vi "Power On Dut.vi"(7 "measure call context in":refnum<class "Measure Call Context.lvclass">, 8 "error in":errorcluster, 11 "Power sequencing file path":path) -> (0 "error out":errorcluster, 5 "measure call context out":refnum<class "Measure Call Context.lvclass">)   [LabVIEW 2023]
uses:
  <vilib>/Plug-In SDKs/Measurements/Measure Call Context/Measure Call Context.lvclass
  NI gRPC Device Server - Action.ctl
  <instrlib>/niDCPower/nidcpower.llb/niDCPower gRPC Device Server.ctl
  <instrlib>/niDCPower/nidcpower.llb/niDCPower Source Mode.ctl
  <instrlib>/niDCPower/nidcpower.llb/niDCPower Output Function.ctl
  <instrlib>/niDigital/niDigital.llb/niDigital gRPC Device Server.ctl
  <instrlib>/niDigital/niDigital.llb/niDigital Output Function.ctl
  <instrlib>/niDigital/niDigital.llb/niDigital PMU Aperture Time Units.ctl
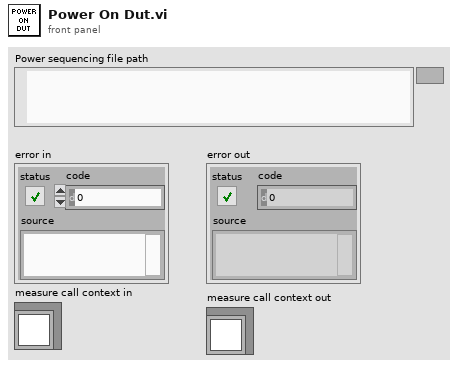
[diagram p1: front panel]
types:
  T1 = typedef "NI gRPC Device Server - Action.ctl" = enum16{"Start Server", "End Server"}
  T2 = typedef "DC Ins Initialize.ctl" = cluster{"Pin Name":string, "Resource Name":refnum<k15>, "Channel":string, "Voltage Range (V)":dbl, "Current Range (A)":dbl, "Instrument Type":T3}
  T3 = typedef "DC Ins Type.ctl" = enum16{"niDigital", "niDCPower", "undefined"}
  T4 = typedef "DC Settings.ctl" = cluster{"Pin Name":string, "Resource Name":refnum<k15>, "Channel":string, "Power-up Seq":u32, "Power-up Voltage (V)":dbl, "Power-down Seq":u32, "Power-down Voltage (V)":dbl, "Current Limit (A)":dbl, "Wait Before Next (ms)":u32, "Instrument Type":T3}
  T5 = typedef "niDCPower gRPC Device Server.ctl" = cluster{"session name":string, "address (localhost)":string, "port (31763)":u32}
  T6 = typedef "niDigital gRPC Device Server.ctl" = cluster{"session name":string, "address (localhost)":string, "port (31763)":u32}
  T7 = typedef "niDCPower Output Function.ctl" = i32
  T8 = typedef "niDCPower Source Mode.ctl" = i32
  T9 = typedef "niDigital PMU Aperture Time Units.ctl" = i32
  T10 = typedef "niDigital Output Function.ctl" = i32
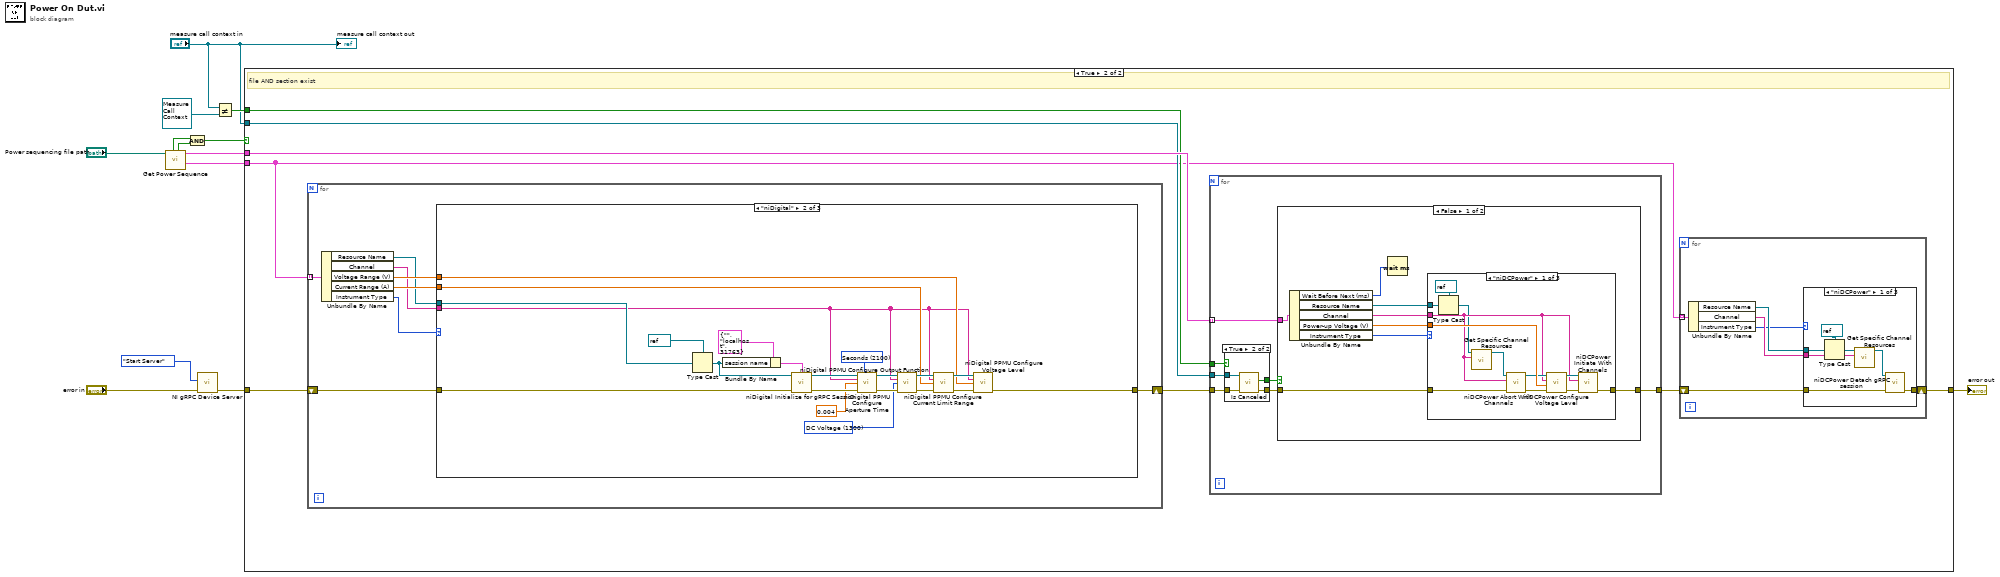
[diagram p0: block diagram]
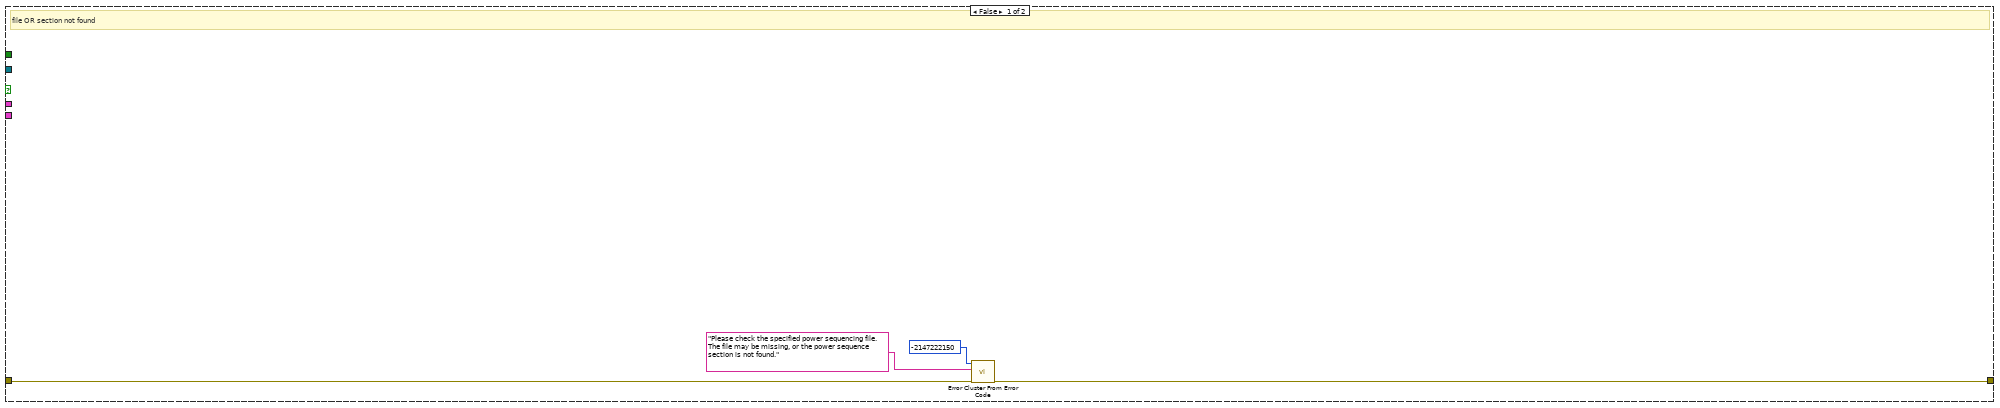
[diagram p2: hidden frame]
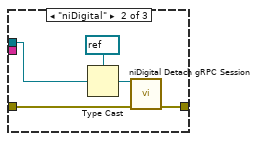
[diagram p3: hidden frame]
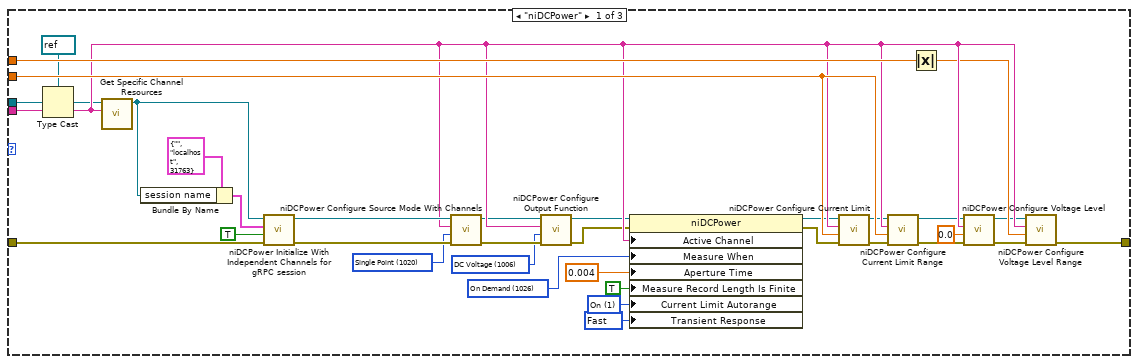
[diagram p5: hidden frame]
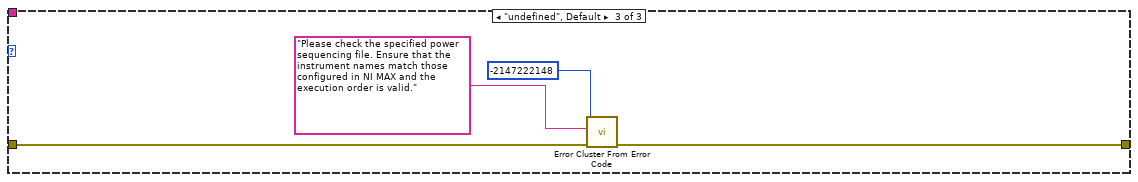
[diagram p6: hidden frame]
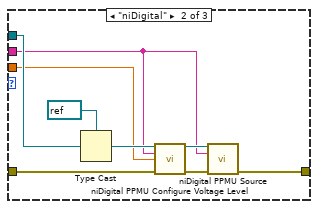
[diagram p8: hidden frame]
diagram:
  n1 = call "Get Power Sequence.vi"("File Path"="Power sequencing file path") -> ("SMUs to Initialize (not in order)"=w12:T2[], "Power up Seq"=w11:T4[], "File Exists?"=w7:bool, "Section Exists?"=w6:bool)  [unwired: 6 in, 1 out]
  n2 = And(x=w6, y=w7) -> (x .and. y?=w8:bool)
  n3 = call "NI gRPC Device Server.vi"("error in"="error in", "Action"=NI_gRPC_Device_Server_-_Action."Start Server") -> ("error out"=w5:errorcluster)  [unwired: 9 in]
  n4 = Not Equal?(x="measure call context in", y=refnum<class "Measure Call Context.lvclass"> refnum ("measure call context in")) -> (x != y?=w4:bool)
  n5 = case shown="True" w8 {
    tunnel: w12 -> [_ w18]
    tunnel: w11 -> [_ w25]
    tunnel: [w17 w21] -> w10
    tunnel: w5 -> [w16 w23]
    tunnel: "measure call context in" -> [_ w20]
    tunnel: w4 -> [_ w19]
    frame False {
      # "file OR section not found"
      n6 = call <vilib>:"Error Cluster From Error Code.vi"("error in (no error)"=w16, "error message (\"\")"="Please check the specified power sequencing file. The file may be missing, or the power sequence section is not found.", "error code (0)"=-2147222150) -> ("error out"=w17:errorcluster)  [unwired: 6 in]
    }
    frame True {
      # "file AND section exist"
      n7 = for {
        tunnel: w18 -> [w51] mode=indexing
        shift-right: [w47] -> w24
        shift-left: w23 -> [w52]
        n8 = Unbundle By Name(w51) -> ("Resource Name"=w46:refnum<k15>, "Channel"=w48:string, "Voltage Range (V)"=w50:dbl, "Current Range (A)"=w49:dbl, "Instrument Type"=w45:T3)
        n9 = case shown="\"niDigital\"" w45 {
          tunnel: w46 -> [w87 w91 _]
          tunnel: w52 -> [w86 w108 w112]
          tunnel: w50 -> [w85 w90 _]
          tunnel: w49 -> [w84 w89 _]
          tunnel: w48 -> [w76 w88 _]
          tunnel: [w83 w107 w111] -> w47
          frame "niDCPower" {
            w53 = 1039 items=["Slow"=1041, "Normal"=1038, "Fast"=1039, "Custom"=1042] ("Source:Transient Response")
            w54 = 1 items=["Off", "On"] ("Measurement:Autorange")
            w69 = 1026 items=["Automatically after Source Complete"=1025, "On Demand"=1026, "On Measure Trigger"=1027] ("Measurement:Advanced:Measure When")
            w70 = T7 1006 items=["DC Voltage"=1006, "DC Current"=1007, "Pulse Voltage"=1049, "Pulse Current"=1050] ("output function")
            w71 = T8 1020 items=["Single Point"=1020, "Sequence"=1021] ("source mode")
            n10 = Type Cast(type=refnum<k15> refnum ("Resource Name"), x=w87) -> (*(type *) &x=w75:refnum<k15>)
            n11 = call "Get Specific Channel Resources.vi"("Channel"=w76, "Resource Name"=w75) -> ("Resource Name"=w77:refnum<k15>)  [unwired: 9 in]
            n12 = Bundle By Name(cluster=T5 {"session name"="", "address (localhost)"="localhost", "port (31763)"=31763} ("gRPC options"), "session name"=w77) -> (w78:T5)
            n13 = call <instrlib>:"niDCPower Initialize With Independent Channels for gRPC session.vi"("error in (no error)"=w86, "reset (false)"=TRUE, "gRPC options"=w78, "resource name"=w77) -> ("error out"=w80:errorcluster, "instrument handle out"=w81:refnum<k15>)  [unwired: 6 in]
            n14 = call <instrlib>:"niDCPower Configure Source Mode With Channels.vi"("error in (no error)"=w80, "source mode"=w71, "channel name"=w76, "instrument handle"=w81) -> ("error out"=w72:errorcluster, "instrument handle out"=w73:refnum<k15>)  [unwired: 6 in]
            n15 = call <instrlib>:"niDCPower Configure Output Function.vi"("error in (no error)"=w72, "output function"=w70, "channel name"=w76, "instrument handle"=w73) -> ("error out"=w65:errorcluster, "instrument handle out"=w66:refnum<k15>)  [unwired: 6 out]
            n16 = property class="niDCPower"(reference=w66, error in=w65, "Active Channel"=w76, "Measure When"=w69, "Aperture Time"=0.004 ("Measurement:Aperture Time"), "Measure Record Length Is Finite"=TRUE ("Measurement:Measure Record Length Is Finite"), "Current Limit Autorange"=w54, "Transient Response"=w53) -> (reference out=w62:refnum<k15>, error out=w61:errorcluster)
            n17 = call <instrlib>:"niDCPower Configure Current Limit.vi"("error in (no error)"=w61, "current limit"=w84, "channel name"=w76, "instrument handle"=w62) -> ("error out"=w59:errorcluster, "instrument handle out"=w60:refnum<k15>)  [unwired: 1 in, 5 out]
            n18 = call <instrlib>:"niDCPower Configure Current Limit Range.vi"("error in (no error)"=w59, "current limit range"=w84, "channel name"=w76, "instrument handle"=w60) -> ("error out"=w57:errorcluster, "instrument handle out"=w58:refnum<k15>)  [unwired: 6 out]
            n19 = Absolute Value(x=w85) -> (abs(x)=w64:dbl)
            n20 = call <instrlib>:"niDCPower Configure Voltage Level.vi"("error in (no error)"=w57, "voltage level"=0.0, "channel name"=w76, "instrument handle"=w58) -> ("error out"=w55:errorcluster, "instrument handle out"=w56:refnum<k15>)  [unwired: 6 in]
            n21 = call <instrlib>:"niDCPower Configure Voltage Level Range.vi"("error in (no error)"=w55, "voltage level range"=w64, "channel name"=w76, "instrument handle"=w56) -> ("error out"=w83:errorcluster)  [unwired: 7 out]
          }
          frame "niDigital" {
            w92 = T9 2100 items=["Seconds"=2100] ("aperture time units")
            w94 = T10 1300 items=["DC Voltage"=1300, "DC Current"=1301] ("output function")
            n22 = Type Cast(type=refnum<k15> refnum ("instrument handle"), x=w91) -> (*(type *) &x=w102:refnum<k15>)
            n23 = Bundle By Name(cluster=T6 {"session name"="", "address (localhost)"="localhost", "port (31763)"=31763} ("gRPC options"), "session name"=w102) -> (w106:T6)
            n24 = call <instrlib>:"niDigital Initialize for gRPC Session.vi"("resource name"=w102, "gRPC options"=w106, "error in"=w108) -> ("instrument handle"=w103:refnum<k15>, "error out"=w104:errorcluster)  [unwired: 11 in]
            n25 = call <instrlib>:"niDigital PPMU Configure Aperture Time.vi"("instrument handle"=w103, "aperture time units"=w92, "channel list"=w88, "aperture time"=0.004 ("Measurement:Aperture Time"), "error in"=w104) -> ("instrument handle out"=w97:refnum<k15>, "error out"=w98:errorcluster)  [unwired: 9 in]
            n26 = call <instrlib>:"niDigital PPMU Configure Output Function.vi"("instrument handle"=w97, "channel list"=w88, "output function"=w94, "error in"=w98) -> ("instrument handle out"=w96:refnum<k15>, "error out"=w99:errorcluster)  [unwired: 10 in]
            n27 = call <instrlib>:"niDigital PPMU Configure Current Limit Range.vi"("instrument handle"=w96, "channel list"=w88, "current limit range (A)"=w89, "error in"=w99) -> ("instrument handle out"=w95:refnum<k15>, "error out"=w100:errorcluster)  [unwired: 10 in]
            n28 = call <instrlib>:"niDigital PPMU Configure Voltage Level.vi"("instrument handle"=w95, "channel list"=w88, "voltage level (V)"=w90, "error in"=w100) -> ("error out"=w107:errorcluster)  [unwired: 10 in, 1 out]
          }
          frame "undefined", Default {
            n29 = call <vilib>:"Error Cluster From Error Code.vi"("error in (no error)"=w112, "error message (\"\")"="Please check the specified power sequencing file. Ensure that the instrument names match those configured in NI MAX and the execution order is valid." ("error message (\"\")"), "error code (0)"=-2147222148) -> ("error out"=w111:errorcluster)  [unwired: 6 in]
          }
        }
      }
      n30 = for {
        tunnel: w25 -> [w119] mode=indexing
        tunnel: w24 -> [w116]
        tunnel: [w118] -> w22
        tunnel: w20 -> [w114]
        tunnel: w19 -> [w113]
        n31 = case shown="True" w113 {
          tunnel: [_ w124] -> w117
          tunnel: w116 -> [w120 w123]
          tunnel: [w120 w122] -> w115
          tunnel: w114 -> [_ w121]
          frame False {
          }
          frame True {
            n32 = call <vilib>:"Is Canceled.vi"("error in"=w123, "measure call context in"=w121) -> ("error out"=w122:errorcluster, "is canceled?"=w124:bool)  [unwired: 7 in, 1 out]
          }
        }
        n33 = case shown="False" w117 {
          tunnel: w119 -> [w131 _]
          tunnel: w115 -> [w129 w155]
          tunnel: [w127 w155] -> w118
          frame False {
            n34 = Unbundle By Name(w131) -> ("Wait Before Next (ms)"=w132:u32, "Resource Name"=w126:refnum<k15>, "Channel"=w128:string, "Power-up Voltage (V)"=w130:dbl, "Instrument Type"=w125:T3)
            n35 = Wait (ms)(milliseconds to wait=w132) -> ()  [unwired: 1 out]
            n36 = case shown="\"niDCPower\"" w125 {
              tunnel: w126 -> [w144 w148 _]
              tunnel: w130 -> [w141 w147 _]
              tunnel: w129 -> [w139 w149 w154]
              tunnel: w128 -> [w136 w146 _]
              tunnel: [w135 w145 w154] -> w127
              frame "niDCPower" {
                n37 = Type Cast(type=refnum<k15> refnum ("Resource Name"), x=w144) -> (*(type *) &x=w134:refnum<k15>)
                n38 = call "Get Specific Channel Resources.vi"("Channel"=w136, "Resource Name"=w134) -> ("Resource Name"=w143:refnum<k15>)  [unwired: 9 in]
                n39 = call <instrlib>:"niDCPower Abort With Channels.vi"("error in (no error)"=w139, "channel name"=w136, "instrument handle"=w143) -> ("error out"=w137:errorcluster, "instrument handle out"=w138:refnum<k15>)  [unwired: 7 in]
                n40 = call <instrlib>:"niDCPower Configure Voltage Level.vi"("error in (no error)"=w137, "voltage level"=w141, "channel name"=w136, "instrument handle"=w138) -> ("error out"=w140:errorcluster, "instrument handle out"=w142:refnum<k15>)  [unwired: 6 in]
                n41 = call <instrlib>:"niDCPower Initiate With Channels.vi"("error in (no error)"=w140, "channel name"=w136, "instrument handle"=w142) -> ("error out"=w135:errorcluster)  [unwired: 7 in, 1 out]
              }
              frame "niDigital" {
                n42 = Type Cast(type=refnum<k15> refnum ("instrument handle"), x=w148) -> (*(type *) &x=w152:refnum<k15>)
                n43 = call <instrlib>:"niDigital PPMU Configure Voltage Level.vi"("instrument handle"=w152, "channel list"=w146, "voltage level (V)"=w147, "error in"=w149) -> ("instrument handle out"=w150:refnum<k15>, "error out"=w151:errorcluster)  [unwired: 10 in]
                n44 = call <instrlib>:"niDigital PPMU Source.vi"("instrument handle"=w150, "channel list"=w146, "error in"=w151) -> ("error out"=w145:errorcluster)  [unwired: 11 in, 1 out]
              }
              frame "undefined", Default {
              }
            }
          }
          frame True {
          }
        }
      }
      n45 = for {
        shift-right: [w30] -> w21
        shift-left: w22 -> [w31]
        tunnel: w18 -> [w29] mode=indexing
        n46 = Unbundle By Name(w29) -> ("Resource Name"=w27:refnum<k15>, "Channel"=w28:string, "Instrument Type"=w26:T3)
        n47 = case shown="\"niDCPower\"" w26 {
          tunnel: w31 -> [w38 w41 w44]
          tunnel: [w37 w40 w44] -> w30
          tunnel: w27 -> [w32 w39 _]
          tunnel: w28 -> [w35 _ _]
          frame "niDCPower" {
            n48 = Type Cast(type=refnum<k15> refnum ("Resource Name"), x=w32) -> (*(type *) &x=w33:refnum<k15>)
            n49 = call "Get Specific Channel Resources.vi"("Channel"=w35, "Resource Name"=w33) -> ("Resource Name"=w36:refnum<k15>)  [unwired: 9 in]
            n50 = call <instrlib>:"niDCPower Detach gRPC session.vi"("error in (no error)"=w38, "instrument handle"=w36) -> ("error out"=w37:errorcluster)  [unwired: 9 in]
          }
          frame "niDigital" {
            n51 = Type Cast(type=refnum<k15> refnum ("instrument handle"), x=w39) -> (*(type *) &x=w42:refnum<k15>)
            n52 = call <instrlib>:"niDigital Detach gRPC Session.vi"("instrument handle"=w42, "error in"=w41) -> ("error out"=w40:errorcluster)  [unwired: 13 in]
          }
          frame "undefined", Default {
          }
        }
      }
    }
  }
  "error out" <- w10
  "measure call context out" <- "measure call context in"
